vi "BncCore.vi"(8 "error in":errorcluster, 9 "queue error in":errorcluster, 10 "queue in":refnum<queue>, 11 "VISA resource":refnum<visa-resource-name>) -> (0 "error out":errorcluster, 2 "queue out":refnum<queue>)   [LabVIEW 2013]
uses:
  BNC_States.ctl
  Command/Set C-Input.ctl
  Command/Set C-Mode.ctl
  Command/Set C-Output.ctl
  Command/Set C-Enable.ctl
  <vilib>/Utility/error.llb/DialogType.ctl
  <instrlib>/BNC/Public/Configure/Configure Sys (To) Mode (Single Shot).vi
  <instrlib>/BNC/Public/Configure/Configure Sys (To) Mode (Normal).vi
  <instrlib>/BNC/Public/Configure/Configure Sys (To) Mode (Duty Cycle).vi
  <instrlib>/BNC/Public/Configure/Configure Sys (To) Mode (Burst).vi
  <instrlib>/BNC/Public/Configure/Configure Chan Mode (Normal).vi
  <instrlib>/BNC/Berkeley Nucleonics 500 Series.lvlib
  <userlib>/Utility/ErrorLog_lib.lvlib
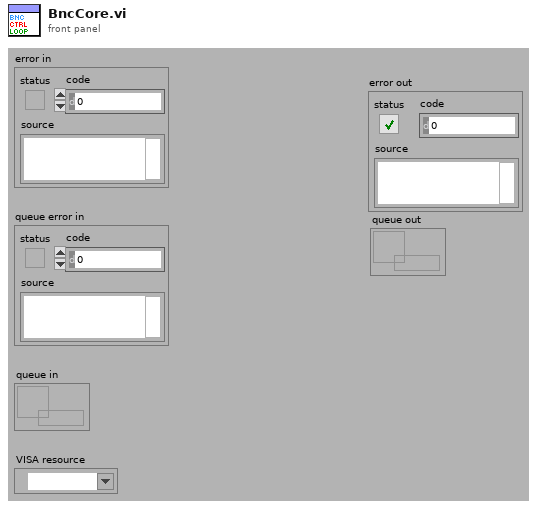
[diagram p1: front panel]
types:
  T1 = cluster{"Rep.Rate":dbl, "Sys Ext Mode":enum16{"Disabled", "Triggered", "Gated", "Triggered & Gated"}, "Mode":enum16{"Normal", "Single Shot", "Duty Cycle", "Burst"}}
  T2 = enum16{"Disabled", "Pulse Inhibit", "Output Inhibit", "Channel"}
  T3 = typedef "Set C-Input.ctl" = cluster{"Channel":i32, "Sync Source":i32}
  T4 = typedef "Set C-Mode.ctl" = cluster{"Channel":i32, "Delay":dbl, "Width":dbl}
  T5 = typedef "Set C-Output.ctl" = cluster{"Channel":i32, "Polarity":bool}
  T6 = typedef "Set C-Enable.ctl" = cluster{"Channel":i32, "Enable":bool}
  T7 = typedef "BNC_States.ctl" = cluster{"State":enum16{"Initialize", "Set System", "Set C-Input", "Set C-Mode", "Set C-Output", "Set C-Enable", "Manl_Trig", "Run", "Stop", "Query C Number", "Close", "Quit"}, "Para.":variant}
  T8 = enum16{"Initialize", "Set System", "Set C-Input", "Set C-Mode", "Set C-Output", "Set C-Enable", "Manl_Trig", "Run", "Stop", "Query C Number", "Close", "Quit"}
  T9 = enum16{"Normal", "Single Shot", "Duty Cycle", "Burst"}
  T10 = enum16{"Disabled", "Triggered", "Gated", "Triggered & Gated"}
  T11 = typedef "DialogType.ctl" = u16
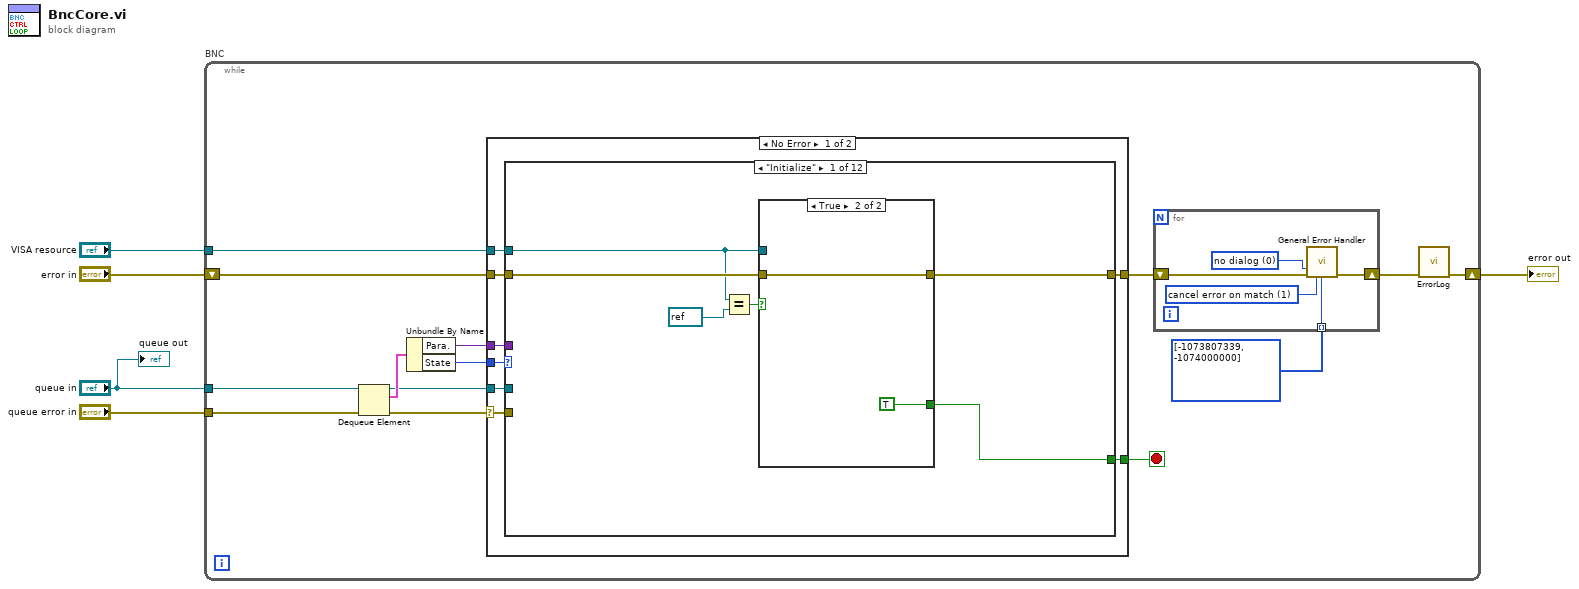
[diagram p0: block diagram]
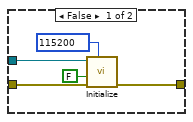
[diagram p2: hidden frame]
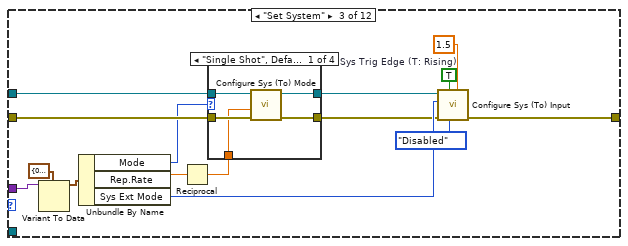
[diagram p4: hidden frame]
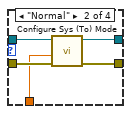
[diagram p5: hidden frame]
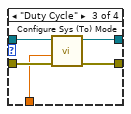
[diagram p6: hidden frame]
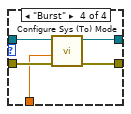
[diagram p7: hidden frame]
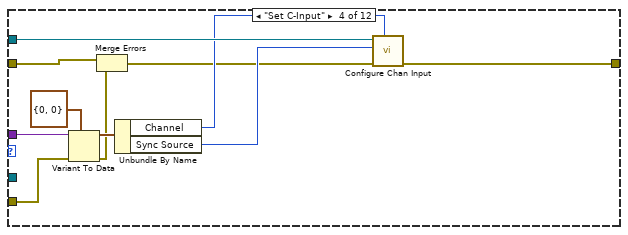
[diagram p8: hidden frame]
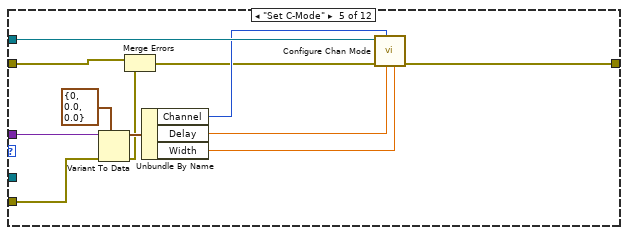
[diagram p9: hidden frame]
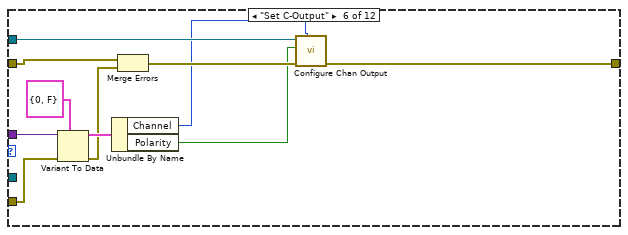
[diagram p10: hidden frame]
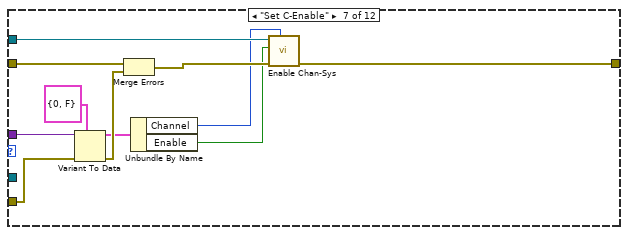
[diagram p11: hidden frame]
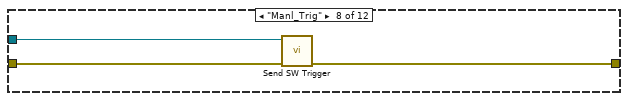
[diagram p12: hidden frame]
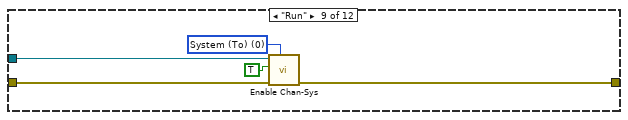
[diagram p13: hidden frame]
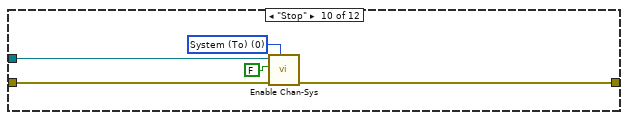
[diagram p14: hidden frame]
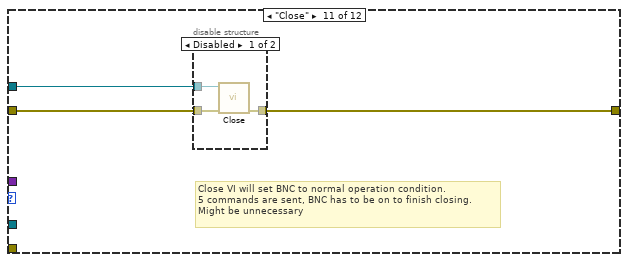
[diagram p15: hidden frame]
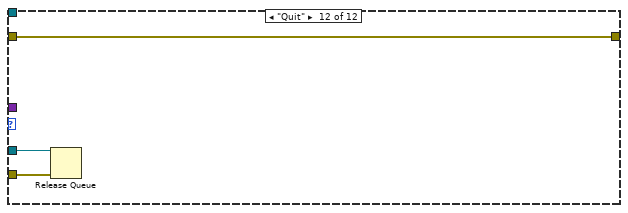
[diagram p17: hidden frame]
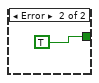
[diagram p18: hidden frame]
diagram:
  n1 = while "BNC" {
    tunnel: "queue in" -> [w19]
    tunnel: "VISA resource" -> [w14]
    shift-right: [w6] -> w1
    shift-left: "error in" -> [w9]
    tunnel: "queue error in" -> [w10]
    stop <- w11 stop-if-true
    n2 = Dequeue Element(queue=w19, error in (no error)=w10) -> (queue out=w15:refnum<queue>, element=w18:T7, error out=w12:errorcluster)  [unwired: 1 in, 1 out]
    n3 = Unbundle By Name(w18) -> ("Para."=w16:variant, "State"=w17:T8)
    n4 = case shown="No Error" w12 {
      selector: w12 -> [w27 _]
      tunnel: w17 -> [w32 _]
      tunnel: w16 -> [w31 _]
      tunnel: w15 -> [w30 _]
      tunnel: w14 -> [w29 _]
      tunnel: w9 -> [w28 _]
      tunnel: [w26 _] -> w13
      tunnel: [w25 TRUE] -> w11
      frame No Error {
        n5 = case shown="\"Initialize\"" w32 {
          tunnel: w27 -> [_ _ _ w89 w100 w110 w121 _ _ _ _ w148]
          tunnel: w31 -> [_ _ w56 w90 w103 w111 w123 _ _ _ _ _]
          tunnel: w30 -> [_ _ _ _ _ _ _ _ _ _ _ w149]
          tunnel: w29 -> [w34 _ w60 w91 w104 w115 w125 w127 w132 w137 w141 _]
          tunnel: w28 -> [w38 w46 w61 w82 w93 w107 w126 w129 w133 w138 w142 w147]
          tunnel: [w37 w46 w59 w92 w102 w114 w124 w128 w131 w136 w140 w147] -> w26
          tunnel: [w33 _ _ _ _ _ _ _ _ _ _ _] -> w25
          frame "Initialize" {
            n6 = Equal?(x=w34, y=refnum<visa-resource-name> refnum ("VISA resource")) -> (x = y?=w36:bool)
            n7 = case shown="True" w36 {
              tunnel: w34 -> [w43 _]
              tunnel: w38 -> [w42 w45]
              tunnel: [w41 w45] -> w37
              tunnel: [_ TRUE] -> w33
              frame False {
                w39 = u32 115200 items=["4800"=4600, "9600"=9600, "19200"=19200, "38400"=38400, "57600"=57600, "115200"=115200] ("Baud Rate (115200)")
                n8 = call <instrlib>:"Initialize.vi"("Baud Rate (115200)"=w39, "error in (no error)"=w42, "Reset? (T: Yes)"=FALSE, "VISA resource name"=w43) -> ("error out"=w41:errorcluster)  [unwired: 6 in, 1 out]
              }
              frame True {
              }
            }
          }
          frame "Query C Number" {
          }
          frame "Set System" {
            w55 = TRUE  # Sys Trig Edge (T: Rising)
            n9 = Variant To Data(type=T1 {"Rep.Rate"=0.0, "Sys Ext Mode"=enum."Triggered", "Mode"=enum."Normal"}, Variant=w56) -> (data=w53:T1)  [unwired: 1 in, 1 out]
            n10 = Unbundle By Name(w53) -> ("Mode"=w49:T9, "Rep.Rate"=w51:dbl, "Sys Ext Mode"=w52:T10)
            n11 = Reciprocal(x=w51) -> (1/x=w50:dbl)
            n12 = case shown="\"Single Shot\", Default" w49 {
              tunnel: w61 -> [w66 w71 w76 w81]
              tunnel: w60 -> [w65 w70 w75 w80]
              tunnel: [w64 w69 w74 w79] -> w48
              tunnel: [w63 w68 w73 w78] -> w58
              tunnel: w50 -> [w62 w67 w72 w77]
              frame "Single Shot", Default {
                n13 = call-poly <instrlib>:"Configure Sys (To) Mode.vi"("error in (no error)"=w66, "Period (100 msec)"=w62, "VISA resource name"=w65) -> ("error out"=w64:errorcluster, "VISA resource name out"=w63:refnum<visa-resource-name>)  [unwired: 7 in]
              }
              frame "Normal" {
                n14 = call-poly <instrlib>:"Configure Sys (To) Mode.vi"("error in (no error)"=w71, "Period (100 msec)"=w67, "VISA resource name"=w70) -> ("error out"=w69:errorcluster, "VISA resource name out"=w68:refnum<visa-resource-name>)  [unwired: 7 in]
              }
              frame "Duty Cycle" {
                n15 = call-poly <instrlib>:"Configure Sys (To) Mode.vi"("error in (no error)"=w76, "Period (100 msec)"=w72, "VISA resource name"=w75) -> ("error out"=w74:errorcluster, "VISA resource name out"=w73:refnum<visa-resource-name>)  [unwired: 7 in]
              }
              frame "Burst" {
                n16 = call-poly <instrlib>:"Configure Sys (To) Mode.vi"("error in (no error)"=w81, "Period (100 msec)"=w77, "VISA resource name"=w80) -> ("error out"=w79:errorcluster, "VISA resource name out"=w78:refnum<visa-resource-name>)  [unwired: 7 in]
              }
            }
            n17 = call <instrlib>:"Configure Sys (To) Input.vi"("Sys Trig Lev (2.5)"=1.5, "Sys Gate Mode"=T2."Disabled", "Sys Trig Edge (T: Rising)"=w55, "error in (no error)"=w48, "Sys Ext Mode"=w52, "VISA resource name"=w58) -> ("error out"=w59:errorcluster)  [unwired: 4 in, 1 out]
          }
          frame "Set C-Input" {
            n18 = Variant To Data(error in=w89, type=T3 {"Channel"=0, "Sync Source"=0} ("cluster"), Variant=w90) -> (data=w87:T3, error out=w84:errorcluster)
            n19 = Merge Errors(w82, w84) -> (w83:errorcluster)
            n20 = Unbundle By Name(w87) -> ("Channel"=w86:i32, "Sync Source"=w85:i32)
            n21 = call <instrlib>:"Configure Chan Input.vi"("Channel (1:Chan A)"=w86, "error in (no error)"=w83, "Sync Source (0:To)"=w85, "VISA resource name"=w91) -> ("error out"=w92:errorcluster)  [unwired: 6 in, 1 out]
          }
          frame "Set C-Mode" {
            n22 = Variant To Data(error in=w100, type=T4 {"Channel"=0, "Delay"=0.0, "Width"=0.0} ("cluster"), Variant=w103) -> (data=w99:T4, error out=w95:errorcluster)
            n23 = Merge Errors(w93, w95) -> (w94:errorcluster)
            n24 = Unbundle By Name(w99) -> ("Channel"=w98:i32, "Delay"=w97:dbl, "Width"=w96:dbl)
            n25 = call-poly <instrlib>:"Configure Chan Mode.vi"("Width (10 msec)"=w96, "Delay (10 msec)"=w97, "Channel (1:Chan A)"=w98, "error in (no error)"=w94, "VISA resource name"=w104) -> ("error out"=w102:errorcluster)  [unwired: 5 in, 1 out]
          }
          frame "Set C-Output" {
            n26 = Variant To Data(error in=w110, type=T5 {"Channel"=0, "Polarity"=FALSE} ("cluster"), Variant=w111) -> (data=w113:T5, error out=w109:errorcluster)
            n27 = Unbundle By Name(w113) -> ("Channel"=w106:i32, "Polarity"=w105:bool)
            n28 = Merge Errors(w107, w109) -> (w108:errorcluster)
            n29 = call <instrlib>:"Configure Chan Output.vi"("Channel (1:Chan A)"=w106, "error in (no error)"=w108, "Polarity (F:Normal)"=w105, "VISA resource name"=w115) -> ("error out"=w114:errorcluster)  [unwired: 6 in, 1 out]
          }
          frame "Set C-Enable" {
            n30 = Variant To Data(error in=w121, type=T6 {"Channel"=0, "Enable"=FALSE} ("cluster"), Variant=w123) -> (data=w118:T6, error out=w120:errorcluster)
            n31 = Merge Errors(w126, w120) -> (w119:errorcluster)
            n32 = Unbundle By Name(w118) -> ("Channel"=w116:i32, "Enable"=w117:bool)
            n33 = call <instrlib>:"Enable Chan-Sys.vi"("Channel (1:Chan A)"=w116, "error in (no error)"=w119, "State (T:Enabled)"=w117, "VISA resource name"=w125) -> ("error out"=w124:errorcluster)  [unwired: 6 in, 1 out]
          }
          frame "Manl_Trig" {
            n34 = call <instrlib>:"Send SW Trigger.vi"("error in (no error)"=w129, "VISA resource name"=w127) -> ("error out"=w128:errorcluster)  [unwired: 8 in, 1 out]
          }
          frame "Run" {
            w134 = 0 items=["System (To)", "Channel A", "Channel B", "Channel C", "Channel D", "Channel E", "Channel F", "Channel G", "Channel H"] ("Channel (1:Chan A)")
            n35 = call <instrlib>:"Enable Chan-Sys.vi"("Channel (1:Chan A)"=w134, "error in (no error)"=w133, "State (T:Enabled)"=TRUE, "VISA resource name"=w132) -> ("error out"=w131:errorcluster)  [unwired: 6 in, 1 out]
          }
          frame "Stop" {
            w139 = 0 items=["System (To)", "Channel A", "Channel B", "Channel C", "Channel D", "Channel E", "Channel F", "Channel G", "Channel H"] ("Channel (1:Chan A)")
            n36 = call <instrlib>:"Enable Chan-Sys.vi"("Channel (1:Chan A)"=w139, "error in (no error)"=w138, "State (T:Enabled)"=FALSE, "VISA resource name"=w137) -> ("error out"=w136:errorcluster)  [unwired: 6 in, 1 out]
          }
          frame "Close" {
            # "Close VI will set BNC to normal operation condition.\n5 commands are sent, BNC has to be on to finish closing.\nMight be unnecessary"
            n37 = disable-structure shown="Disabled" {
              disable-tunnel: w142 -> [w145 w146]
              disable-tunnel: w141 -> [w144 _]
              disable-tunnel: [w143 w146] -> w140
              frame Disabled {
                n38 = call <instrlib>:"Close.vi"("error in (no error)"=w145, "VISA resource name"=w144) -> ("error out"=w143:errorcluster)  [unwired: 9 in]
              }
              frame Enabled {
              }
            }
          }
          frame "Quit" {
            n39 = Release Queue(queue=w149, error in (no error)=w148) -> ()  [unwired: 1 in, 3 out]
          }
        }
      }
      frame Error {
      }
    }
    n40 = for {
      tunnel: i32[] [-1073807339, -1074000000] -> [w20] mode=indexing
      shift-right: [w21] -> w8
      shift-left: w13 -> [w24]
      w23 = 1 items=["no exception", "cancel error on match", "set error on match"] ("[exception action] (none:0)")
      w22 = T11 0 items=["no dialog", "OK message", "continue or stop message", "OK message + warnings", "continue/stop + warnings"] ("type of dialog (OK msg:1)")
      n41 = call <vilib>:"General Error Handler.vi"("type of dialog (OK msg:1)"=w22, "error in (no error)"=w24, "[exception action] (none:0)"=w23, "[exception code]"=w20) -> ("error out"=w21:errorcluster)  [unwired: 7 in, 4 out]
    }
    n42 = call <userlib>:"ErrorLog.vi"("error in (no error)"=w8) -> ("error out"=w6:errorcluster)  [unwired: 10 in]
  }
  "error out" <- w1
  "queue out" <- "queue in"
